vi "Invoke Interface Method.vi"(8 "error in":errorcluster, 9 "method name":string, 10 "interface name":string, 11 "object in":T1) -> (0 "error out":errorcluster, 2 "value":T1, 3 "object out":T1)   [LabVIEW 2026, in "ToastNotification.lvlib" / "Reflection DotNet.lvlib"]
doc: "Invoke a parameterless method through a named interface on a borrowed .NET object. Acquire and release the object Type, interface Type and MethodInfo. value is the acquired boxed return value; its caller must close it even if an error is returned. Skip invocation on incoming error. Does not close or dispose the input object."
uses:
  Reflection DotNet.lvlib
  Callback Object Reference.ctl
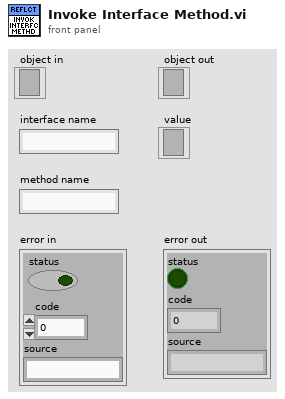
[diagram p1: front panel]
types:
  T1 = typedef "ToastNotification.lvlib/Reflection DotNet.lvlib/Callback Object Reference.ctl" = refnum<k24>
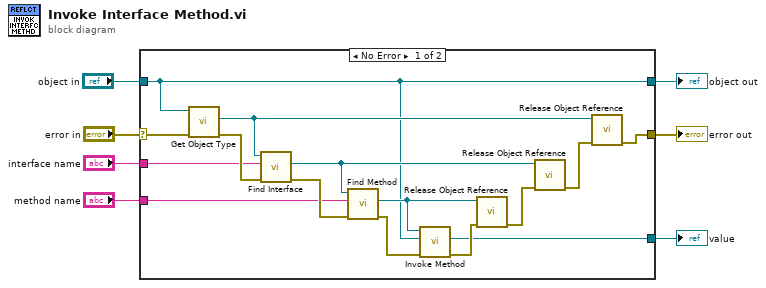
[diagram p0: block diagram]
diagram:
  n1 = case shown="No Error" "error in" {
    selector: "error in" -> [w9 w24]
    tunnel: "object in" -> [w8 w23]
    tunnel: "interface name" -> [w10 _]
    tunnel: "method name" -> [w11 _]
    tunnel: [w18 _] -> w6
    tunnel: [w22 w24] -> w7
    tunnel: [w8 w23] -> w1
    frame No Error {
      n2 = call "Get Object Type.vi"("error in (no error)"=w9, "Object in"=w8) -> ("error out"=w13:errorcluster, "Object Type"=w12:refnum<k24>)  [unwired: 7 in, 1 out]
      n3 = call "Find Interface.vi"("error in (no error)"=w13, "Interface Name"=w10, "Object Type in"=w12) -> ("error out"=w15:errorcluster, "Interface Type"=w14:refnum<k24>)  [unwired: 6 in, 1 out]
      n4 = call "Find Method.vi"("error in (no error)"=w15, "Method Name"=w11, "Declaring Type in"=w14) -> ("error out"=w17:errorcluster, "Method Info"=w16:refnum<k24>)  [unwired: 6 in, 1 out]
      n5 = call "Invoke Method.vi"("error in (no error)"=w17, "Target Object"=w8, "Method Info in"=w16) -> ("error out"=w19:errorcluster, "Return Value"=w18:refnum<k24>)  [unwired: 6 in, 1 out]
      n6 = call "Release Object Reference.vi"("error in"=w19, "object"=w16) -> ("error out"=w20:errorcluster)  [unwired: 9 in]
      n7 = call "Release Object Reference.vi"("error in"=w20, "object"=w14) -> ("error out"=w21:errorcluster)  [unwired: 9 in]
      n8 = call "Release Object Reference.vi"("error in"=w21, "object"=w12) -> ("error out"=w22:errorcluster)  [unwired: 9 in]
    }
    frame Error {
    }
  }
  "value" <- w6
  "error out" <- w7
  "object out" <- w1
